vi "Acquire Data.vi"(7 "user event":T2, 8 "error in":errorcluster, 9 "UI Refs":T1, 10 "Waveforms":waveform(dbl)[](array[waveform]), 11 "4way Leakage":refnum<class "Leakage.lvclass">) -> (0 "error out":errorcluster, 3 "4way Leakage out":refnum<class "Leakage.lvclass">)   [LabVIEW 2025, in "Flow Grind.lvlib" / "Leakage.lvclass"]
uses:
  Leakage.lvclass
  Users/Public/Documents/Sandia National Labs/TSS Plugin/CEF.lvlibp/Node/UserEventRef.ctl
  Users/Public/Documents/Sandia National Labs/TSS Plugin/Tests/XY Plotter.lvlibp/XY  Plotter/XY Plotter.lvclass
  Users/Public/Documents/Sandia National Labs/TSS Plugin/CEF.lvlibp/Node/CEF_Node.lvclass
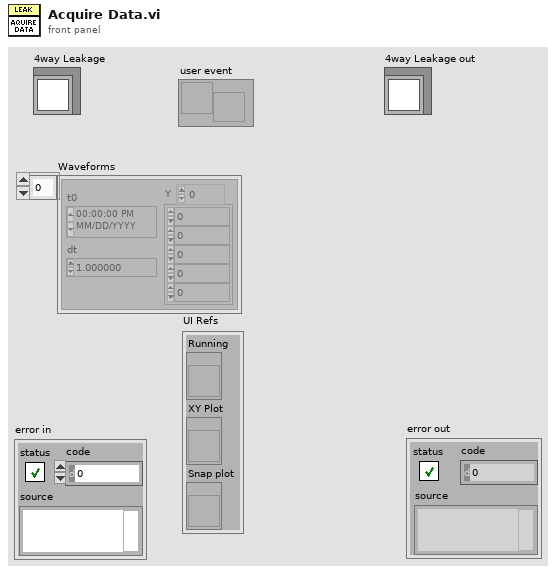
[diagram p1: front panel]
types:
  T1 = cluster{"Running":refnum<vi>, "XY Plot":refnum<vi>, "Snap plot":refnum<vi>}
  T2 = typedef "CEF.lvlibp/CEF_Node.lvclass/UserEventRef.ctl" = refnum<user-event>
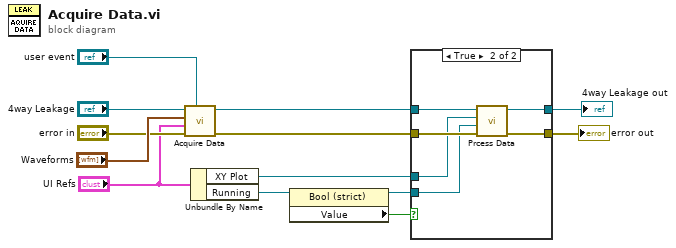
[diagram p0: block diagram]
diagram:
  n1 = call-parent "Acquire Data.vi"("user event"="user event", "error in (no error)"="error in", "UI Refs"="UI Refs", "Waveforms"="Waveforms", "XY Plotter"="4way Leakage") -> ("error out"=w6:errorcluster, "XY Plotter out"=w10:refnum<class "Leakage.lvclass">)  [unwired: 5 in]
  n2 = Unbundle By Name("UI Refs") -> ("XY Plot"=w4:refnum<vi>, "Running"=w3:refnum<vi>)
  n3 = property class="Bool (strict)"(reference=w3) -> (reference out=w1:refnum<vi>, "Value"=w2:bool)  [unwired: 1 in, 1 out]
  n4 = case shown="True" w2 {
    tunnel: w10 -> [w15 w21]
    tunnel: [w15 w20] -> w9
    tunnel: [w14 w18] -> w8
    tunnel: w6 -> [w14 w19]
    tunnel: w4 -> [_ w17]
    tunnel: w1 -> [_ w16]
    frame False {
    }
    frame True {
      n5 = call "Prcess Data.vi"("error in (no error)"=w19, "Running"=w16, "XY Plot"=w17, "Leakage"=w21) -> ("error out"=w18:errorcluster, "Leakage out"=w20:refnum<class "Leakage.lvclass">)  [unwired: 6 in]
    }
  }
  "error out" <- w8
  "4way Leakage out" <- w9
